vi "Add Unicode Header.vi"(2 "Array":string[](array[string]), 3 "Text":string) -> (0 "Array with header 2":string[](array[string]), 1 "Text with header":string)   [LabVIEW 2019, in "Language Selection.lvlib"]
doc: "- - -\nCopyright (c) 2026, Merecs Engineering GmbH"
uses:
  Language Selection.lvlib
panel:
  # "Connector Pane"
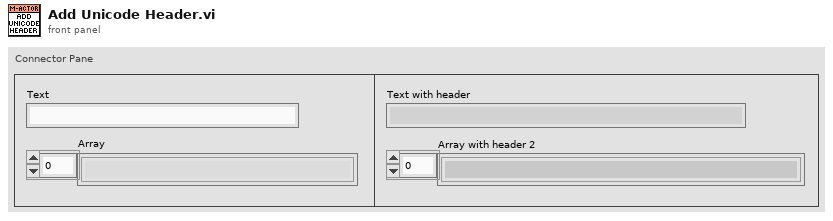
[diagram p1: front panel]
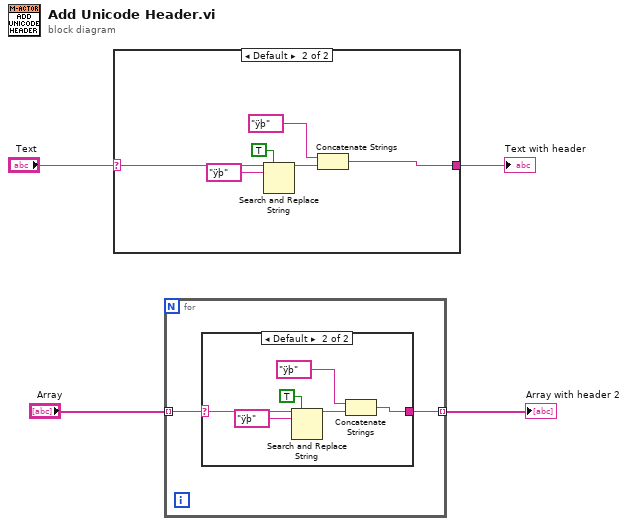
[diagram p0: block diagram]
diagram:
  n1 = case shown="Default" "Text" {
    selector: "Text" -> [w5 w9]
    tunnel: [w5 w11] -> w4
    frame "" {
    }
    frame Default {
      n2 = Search and Replace String(replace all?=TRUE ("replace all? (F)"), input string=w9, search string="ÿþ" ("string")) -> (result string=w6:string)  [unwired: 5 in, 3 out]
      n3 = Concatenate Strings("ÿþ" ("string"), w6) -> (w11:string)
    }
  }
  "Text with header" <- w4
  n4 = for {
    tunnel: "Array" -> [w13] mode=indexing
    tunnel: [w12] -> w1 mode=indexing
    n5 = case shown="Default" w13 {
      selector: w13 -> [w14 w18]
      tunnel: [w14 w20] -> w12
      frame "" {
      }
      frame Default {
        n6 = Search and Replace String(replace all?=TRUE ("replace all? (F)"), input string=w18, search string="ÿþ" ("string")) -> (result string=w15:string)  [unwired: 5 in, 3 out]
        n7 = Concatenate Strings("ÿþ" ("string"), w15) -> (w20:string)
      }
    }
  }
  "Array with header 2" <- w1
